vi "Day 10.vi"() -> ()   [LabVIEW 2021]
uses:
  9d14903f-e169-4f0a-a442-cdeb49079b53.vi
  <vilib>/Utility/file.llb/Read Delimited Spreadsheet (string).vi
  <vilib>/Comparison/Less/Less Functor/Less Functor.lvclass
panel:
  out "Part 1 Solution":i32
  out "input":string[](array[string])
  out "Part 2 Solution":u64
  in  "Input File":enum32{"example input", "input"}(radio)
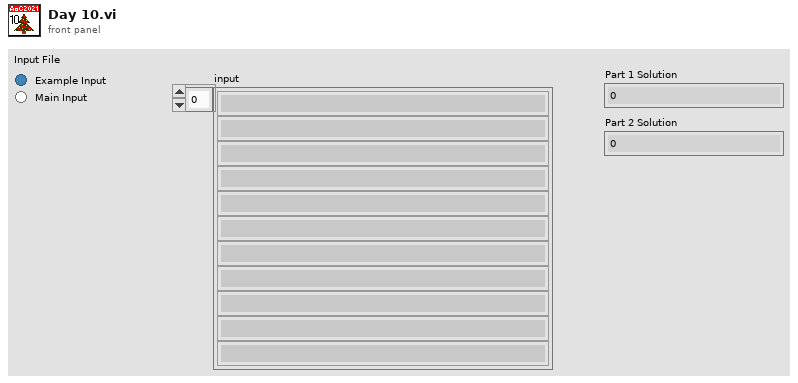
[diagram p1: front panel]
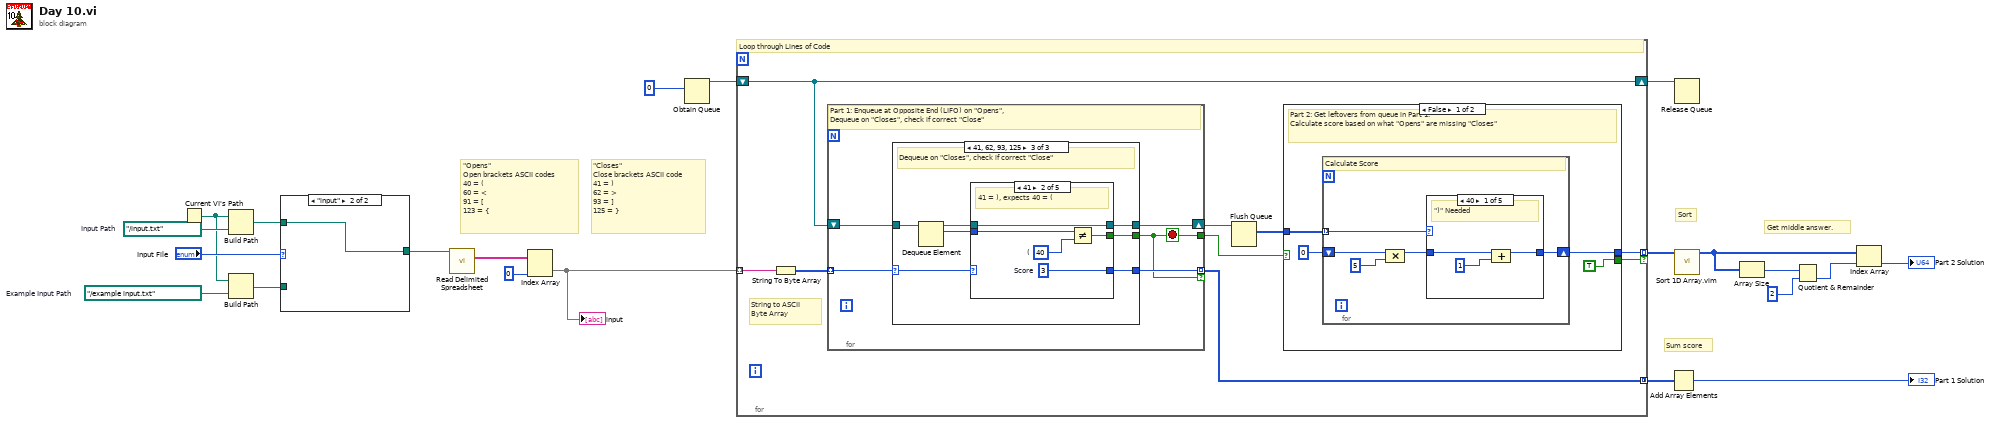
[diagram p0: block diagram]
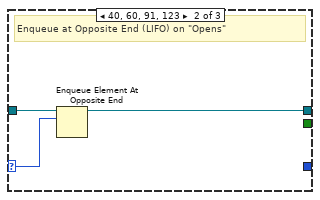
[diagram p4: hidden frame]
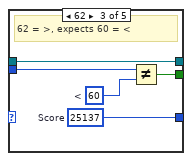
[diagram p6: hidden frame]
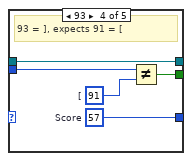
[diagram p7: hidden frame]
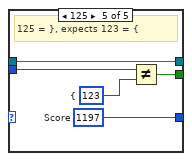
[diagram p8: hidden frame]
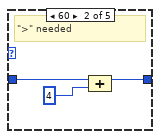
[diagram p9: hidden frame]
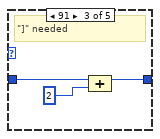
[diagram p10: hidden frame]
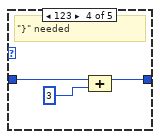
[diagram p11: hidden frame]
diagram:
  w20 = path "../example input.txt"  # Example Input Path
  w21 = path "../input.txt"  # Input Path
  # "Sort"
  # "Sum score"
  # "Get middle answer."
  # "\"Closes\"\nClose brackets ASCII code\n41 = )\n62 = >\n93 = ] \n125 = }"
  # "\"Opens\"\nOpen brackets ASCII codes\n40 = (\n60 = <\n91 = [ \n123 = {"
  n1 = Current VI's Path() -> (path=w15:path)
  n2 = Build Path(base path=w15, name or relative path=w21) -> (appended path=w18:path)
  n3 = Build Path(base path=w15, name or relative path=w20) -> (appended path=w17:path)
  n4 = case shown="\"input\"" "Input File" {
    tunnel: w18 -> [_ w23]
    tunnel: w17 -> [w22 _]
    tunnel: [w22 w23] -> w16
    frame "example input" {
    }
    frame "input" {
    }
  }
  n5 = call-poly <vilib>:"Read Delimited Spreadsheet.vi"("file path (dialog if empty)"=w16) -> ("all rows"=w14:string[][])  [unwired: 9 in, 5 out]
  n6 = Index Array(array=w14, index (col)=0 ("disabled index (col)")) -> (element=w12:string[])  [unwired: 1 in]
  "input" <- w12
  n7 = Obtain Queue(element data type=u8 0) -> (queue out=w10:refnum<queue>)  [unwired: 4 in, 2 out]
  n8 = for {
    tunnel: w12 -> [w31] mode=indexing
    tunnel: [w26] -> w2 mode=indexing if=w25
    tunnel: [w29] -> w3 mode=concatenating
    shift-right: [w24] -> w1
    shift-left: w10 -> [w24]
    # "String to ASCII Byte Array"
    # "Loop through Lines of Code"
    n9 = String To Byte Array(string=w31) -> (unsigned byte array=w32:u8[])
    n10 = for {
      tunnel: w32 -> [w37] mode=indexing
      tunnel: [w36] -> w29 mode=indexing if=w33
      tunnel: [w33] -> w27
      shift-right: [w35] -> w30
      shift-left: w24 -> [w34]
      stop <- w33 stop-if-true
      # "Part 1: Enqueue at Opposite End (LIFO) on \"Opens\", \nDequeue on \"Closes\", check if correct \"Close\""
      n11 = case shown="41, 62, 93, 125" w37 {
        selector: w37 -> [_ w40 w47]
        tunnel: w34 -> [w38 w41 w42]
        tunnel: [_ _ w46] -> w33
        tunnel: [_ _ w45] -> w36
        tunnel: [w38 w39 w43] -> w35
        frame Default {
        }
        frame 40, 60, 91, 123 {
          # "Enqueue at Opposite End (LIFO) on \"Opens\""
          n12 = Enqueue Element At Opposite End(queue=w41, element=w40) -> (queue out=w39:refnum<queue>)  [unwired: 2 in, 2 out]
        }
        frame 41, 62, 93, 125 {
          # "Dequeue on \"Closes\", check if correct \"Close\""
          n13 = Dequeue Element(queue=w42) -> (queue out=w44:refnum<queue>, element=w48:u8)  [unwired: 2 in, 2 out]
          n14 = case shown="41" w47 {
            tunnel: w48 -> [_ w54 w59 w64 w69]
            tunnel: [_ w52 w57 w62 w67] -> w46
            tunnel: [_ w51 w56 w61 w66] -> w45
            tunnel: w44 -> [w49 w50 w55 w60 w65]
            tunnel: [w49 w50 w55 w60 w65] -> w43
            frame 0, Default {
            }
            frame 41 {
              w51 = 3  # Score
              w53 = u8 40  # (
              # "41 = ), expects 40 = ("
              n15 = Not Equal?(x=w54, y=w53) -> (x != y?=w52:bool)
            }
            frame 62 {
              w56 = 25137  # Score
              w58 = u8 60  # <
              # "62 = >, expects 60 = <"
              n16 = Not Equal?(x=w59, y=w58) -> (x != y?=w57:bool)
            }
            frame 93 {
              w61 = 57  # Score
              w63 = u8 91  # [
              # "93 = ], expects 91 = ["
              n17 = Not Equal?(x=w64, y=w63) -> (x != y?=w62:bool)
            }
            frame 125 {
              w66 = 1197  # Score
              w68 = u8 123  # {
              # "125 = }, expects 123 = {"
              n18 = Not Equal?(x=w69, y=w68) -> (x != y?=w67:bool)
            }
          }
        }
      }
    }
    n19 = Flush Queue(queue=w30) -> (remaining elements=w28:u8[])  [unwired: 1 in, 2 out]
    n20 = case shown="False" w27 {
      tunnel: w28 -> [w72 _]
      tunnel: [w71 _] -> w26
      tunnel: [TRUE _] -> w25
      frame False {
        # "Part 2: Get leftovers from queue in Part 1.  \nCalculate score based on what \"Opens\" are missing \"Closes\""
        n21 = for {
          tunnel: w72 -> [w78] mode=indexing
          shift-right: [w74] -> w71
          shift-left: u64 0 -> [w77]
          # "Calculate Score"
          n22 = Compound Arithmetic op=MULTIPLY(w77, u64 5) -> (w75:u64)
          n23 = case shown="40" w78 {
            tunnel: w75 -> [w81 w84 w87 w90 w91]
            tunnel: [w79 w82 w85 w88 w91] -> w74
            frame 40 {
              # "\")\" Needed"
              n24 = Compound Arithmetic op=ADD(w81, u64 1) -> (w79:u64)
            }
            frame 60 {
              # "\">\" needed"
              n25 = Compound Arithmetic op=ADD(w84, u64 4) -> (w82:u64)
            }
            frame 91 {
              # "\"]\" needed"
              n26 = Compound Arithmetic op=ADD(w87, u64 2) -> (w85:u64)
            }
            frame 123 {
              # "\"}\" needed"
              n27 = Compound Arithmetic op=ADD(w90, u64 3) -> (w88:u64)
            }
            frame Default {
            }
          }
        }
      }
      frame True {
        # "Corrupted. Ignore for Part 2"
      }
    }
  }
  n28 = Add Array Elements(numeric array=w3) -> (sum=→"Part 1 Solution":i32)
  n29 = Release Queue(queue=w1) -> ()  [unwired: 2 in, 3 out]
  n30 = call "Sort 1D Array.vim"("unsorted array"=w2) -> ("sorted array"=w5:u64[])  [unwired: 10 in]
  n31 = Array Size(array=w5) -> (size(s)=w7:i32)
  n32 = Quotient & Remainder(x=w7, y=2) -> (floor(x/y)=w4:i32)  [unwired: 1 out]
  n33 = Index Array(array=w5, index=w4) -> (element=→"Part 2 Solution":u64)
